vi "Host_main_Lab8.vi"() -> ()   [LabVIEW 2025]
uses:
  vi/thresholds.ctl
  UI_Msg.ctl
  action.ctl
  states.ctl
panel:
  out "cmd_ok":bool
  in  "Stop RT":bool
  out "Connected?":bool
  in  "IP myRIO":string="172.22.11.2"
  out "error out":errorcluster
  in  "Manual trigger":bool
  in  "parameters":T1
  out "Waveform Graph":i16[][](graph)
  in  "Close":bool
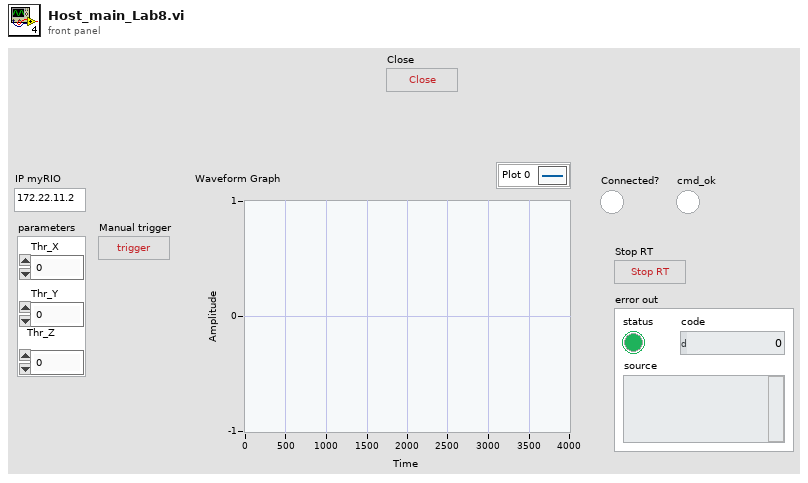
[diagram p1: front panel]
types:
  T1 = typedef "thresholds.ctl" = cluster{"Thr_X":i16, "Thr_Y":i16, "Thr_Z":i16}
  T2 = typedef "states.ctl" = enum16{"Run", "Connect"}
  T3 = typedef "UI_Msg.ctl" = cluster{"action":T4, "Threshold":T1}
  T4 = typedef "action.ctl" = enum16{"Thresholds_Changed", "Manual_Trigger", "Stop"}
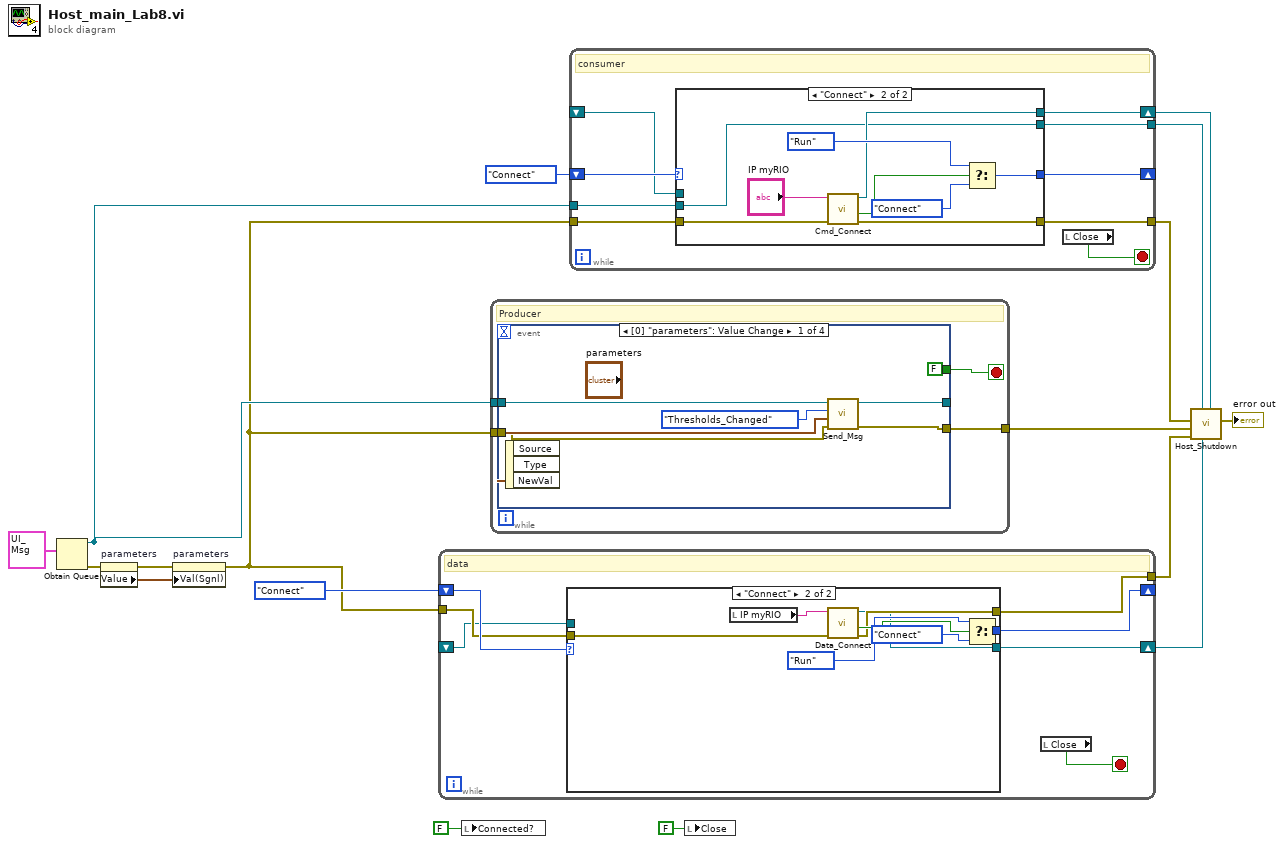
[diagram p0: block diagram]
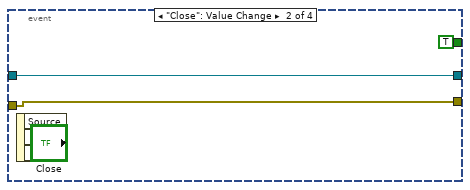
[diagram p2: hidden frame]
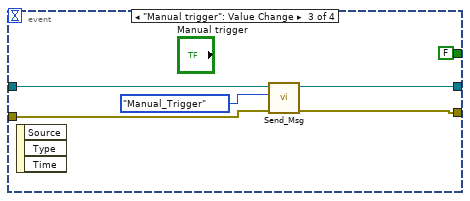
[diagram p3: hidden frame]
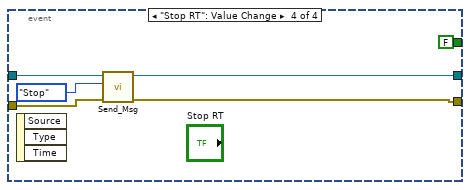
[diagram p4: hidden frame]
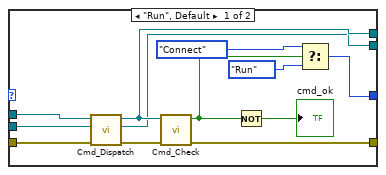
[diagram p5: hidden frame]
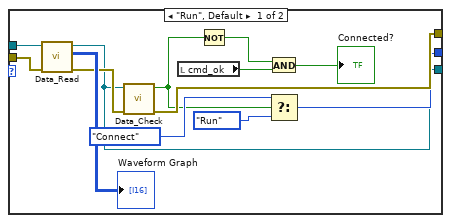
[diagram p6: hidden frame]
diagram:
  n1 = Obtain Queue(element data type=T3 {"action"=enum."Thresholds_Changed", "Threshold"={"Thr_X"=0, "Thr_Y"=0, "Thr_Z"=0}} ("msg")) -> (queue out=w9:refnum<queue>, error out=w11:errorcluster)  [unwired: 4 in, 1 out]
  n2 = property on="parameters" class="Clust (strict)"(error in=w11) -> (error out=w15:errorcluster, "Value"=w14:T1)  [unwired: 1 in, 1 out]
  n3 = property on="parameters" class="Clust (strict)"(error in=w15, "Val(Sgnl)"=w14) -> (error out=w3:errorcluster)  [unwired: 1 in, 1 out]
  n4 = while {
    tunnel: w3 -> [w22]
    shift-right: [w23] -> _
    shift-left: states."Connect" ("Enum") -> [w24]
    tunnel: [w21] -> w2
    shift-right: [w19] -> w1
    shift-left: _ -> [w18]
    stop <- w20 stop-if-true
    # "data"
    n5 = case shown="\"Connect\"" w24 {
      tunnel: [w30 w42] -> w23
      tunnel: w22 -> [w36 w40]
      tunnel: [w33 w39] -> w21
      tunnel: [w29 w38] -> w19
      tunnel: w18 -> [w37 _]
      frame "Run", Default {
        n6 = call "Data_Read.vi"("error in"=w36, "reader ref in"=w37) -> ("error out"=w34:errorcluster, "Array"=→"Waveform Graph":i16[][], "reader ref out"=w29:refnum<k21>)  [unwired: 7 in]
        n7 = call "Data_Check.vi"("error in"=w34, "writer ref in"=w29) -> ("error out"=w33:errorcluster, "disconnected?"=w28:bool)  [unwired: 8 in]
        n8 = local read "cmd_ok"() -> (w26:bool)
        n9 = Not(x=w28) -> (.not. x?=w27:bool)
        n10 = And(x=w27, y=w26) -> (x .and. y?=→"Connected?":bool)
        n11 = Select(t=states."Connect" ("Enum"), s=w28, f=states."Run") -> (s? t:f=w30:T2)
      }
      frame "Connect" {
        n12 = local read "IP myRIO"() -> (w41:string)
        n13 = call "Data_Connect.vi"("error in"=w40, "IP myRIO in"=w41) -> ("error out"=w39:errorcluster, "connected?"=w44:bool, "reader endpoint out"=w38:refnum<k21>)  [unwired: 7 in]
        n14 = Select(t=states."Run" ("Enum"), s=w44, f=states."Connect") -> (s? t:f=w42:T2)
      }
    }
    n15 = local read "Close"() -> (w20:bool)
  }
  n16 = local write "Connected?"(FALSE ("Connected?")) -> ()
  n17 = while {
    tunnel: w3 -> [w48]
    tunnel: w9 -> [w46]
    tunnel: [w47] -> w4
    stop <- w49 stop-if-true
    # "Producer"
    n18 = event shown="[0] \"parameters\": Value Change" {
      selector: _ -> [_ _ _ _]
      dyn-events: _ -> [_ _ _ _]
      timeout: _ -> [_ _ _ _]
      tunnel: [FALSE TRUE FALSE FALSE] -> w49
      tunnel: [w53 w58 w62 w66] -> _
      tunnel: w48 -> [w52 w57 w65 w68]
      tunnel: [w51 w57 w61 w67] -> w47
      tunnel: w46 -> [w54 w58 w64 w69]
      event Value Change {
        n19 = event-data() -> ("NewVal"=w55:T1)  [unwired: 1 in, 2 out]
        n20 = call "Send_Msg.vi"("error in (no error)"=w52, "NewVal"=w55, "action"=action."Thresholds_Changed", "Queue in"=w54) -> ("error out"=w51:errorcluster, "Queue out"=w53:refnum<queue>)  [unwired: 6 in]
      }
      event "Close": Value Change {
        n21 = event-data() -> ()  [unwired: 1 in, 3 out]
      }
      event "Manual trigger": Value Change {
        n22 = event-data() -> ()  [unwired: 1 in, 3 out]
        n23 = call "Send_Msg.vi"("error in (no error)"=w65, "action"=action."Manual_Trigger", "Queue in"=w64) -> ("error out"=w61:errorcluster, "Queue out"=w62:refnum<queue>)  [unwired: 7 in]
      }
      event "Stop RT": Value Change {
        n24 = event-data() -> ()  [unwired: 1 in, 3 out]
        n25 = call "Send_Msg.vi"("error in (no error)"=w68, "action"=action."Stop", "Queue in"=w69) -> ("error out"=w67:errorcluster, "Queue out"=w66:refnum<queue>)  [unwired: 7 in]
      }
    }
  }
  n26 = while {
    shift-right: [w78] -> _
    shift-left: states."Connect" ("Enum") -> [w80]
    tunnel: w3 -> [w79]
    shift-right: [w77] -> w6
    shift-left: _ -> [w76]
    tunnel: w9 -> [w75]
    tunnel: [w73] -> w7
    tunnel: [w72] -> w5
    stop <- w74 stop-if-true
    # "consumer"
    n27 = case shown="\"Connect\"" w80 {
      tunnel: [w84 w96] -> w72
      tunnel: w79 -> [w90 w98]
      tunnel: [w86 w99] -> w78
      tunnel: [w85 w94] -> w77
      tunnel: w76 -> [w92 _]
      tunnel: w75 -> [w91 w93]
      tunnel: [w81 w93] -> w73
      frame "Run", Default {
        n28 = call "Cmd_Dispatch.vi"("error in"=w90, "queue in"=w91, "writer endpoint in"=w92) -> ("error Iout"=w89:errorcluster, "queue out"=w81:refnum<queue>, "writer endpoint out"=w85:refnum<k21>)  [unwired: 6 in]
        n29 = call "Cmd_Check.vi"("error in"=w89, "writer ref in"=w85) -> ("error out"=w84:errorcluster, "disconnected?"=w83:bool)  [unwired: 8 in]
        n30 = Not(x=w83) -> (.not. x?=→"cmd_ok":bool)
        n31 = Select(t=states."Connect" ("Enum"), s=w83, f=states."Run" ("Enum")) -> (s? t:f=w86:T2)
      }
      frame "Connect" {
        n32 = call "Cmd_Connect.vi"("error in (no error)"=w98, "IP myRIO in"="IP myRIO") -> ("error out"=w96:errorcluster, "connected?"=w95:bool, "Refnum out"=w94:refnum<k21>)  [unwired: 7 in]
        n33 = Select(t=states."Run" ("Enum"), s=w95, f=states."Connect") -> (s? t:f=w99:T2)
      }
    }
    n34 = local read "Close"() -> (w74:bool)
  }
  n35 = local write "Close"(FALSE ("Stop")) -> ()
  n36 = call "Host_Shutdown.vi"("writer ref"=w6, "reader ref"=w1, "Queue in"=w7, "error in 2"=w2, "error in 1"=w4, "error in 3"=w5) -> ("error out"=→"error out":errorcluster)  [unwired: 5 in]
